vi "SaveWfmTxtNEW (SubVI).vi"(8 "error in":errorcluster, 11 "АЧХ":cluster{dbl[], dbl[]}[](graph) caption="XY Graph - Light") -> (0 "error out":errorcluster)   [LabVIEW 2017]
uses:
  <vilib>/Utility/file.llb/Write Delimited Spreadsheet (DBL).vi
panel:
  out "output array":dbl[][](array[numeric])
  out "Array":dbl[][](array[numeric])
  out "dt":dbl[](array[numeric])
  out "Y":dbl[](array[numeric])
  in  "Osc":waveform(dbl)[](graph)=[{"t0"=timestamp(0 s since 1904-01-01), "dt"=0.0002500000118743628, "Y"=array[20608 elements]}, {"t0"=timestamp(0 s since 1904-01-01), "dt"=0.0002500000118743628, "Y"=array[20608 elements]}, {"t0"=timestamp(0 s since 1904-01-01), "dt"=0.0002500000118743628, "Y"=array[20608 elements]}, {"t0"=timestamp(0 s since 1904-01-01), "dt"=0.0002500000118743628, "Y"=array[20608 elements]}] caption="Осциллограмма"
  # "Сохранение данных"
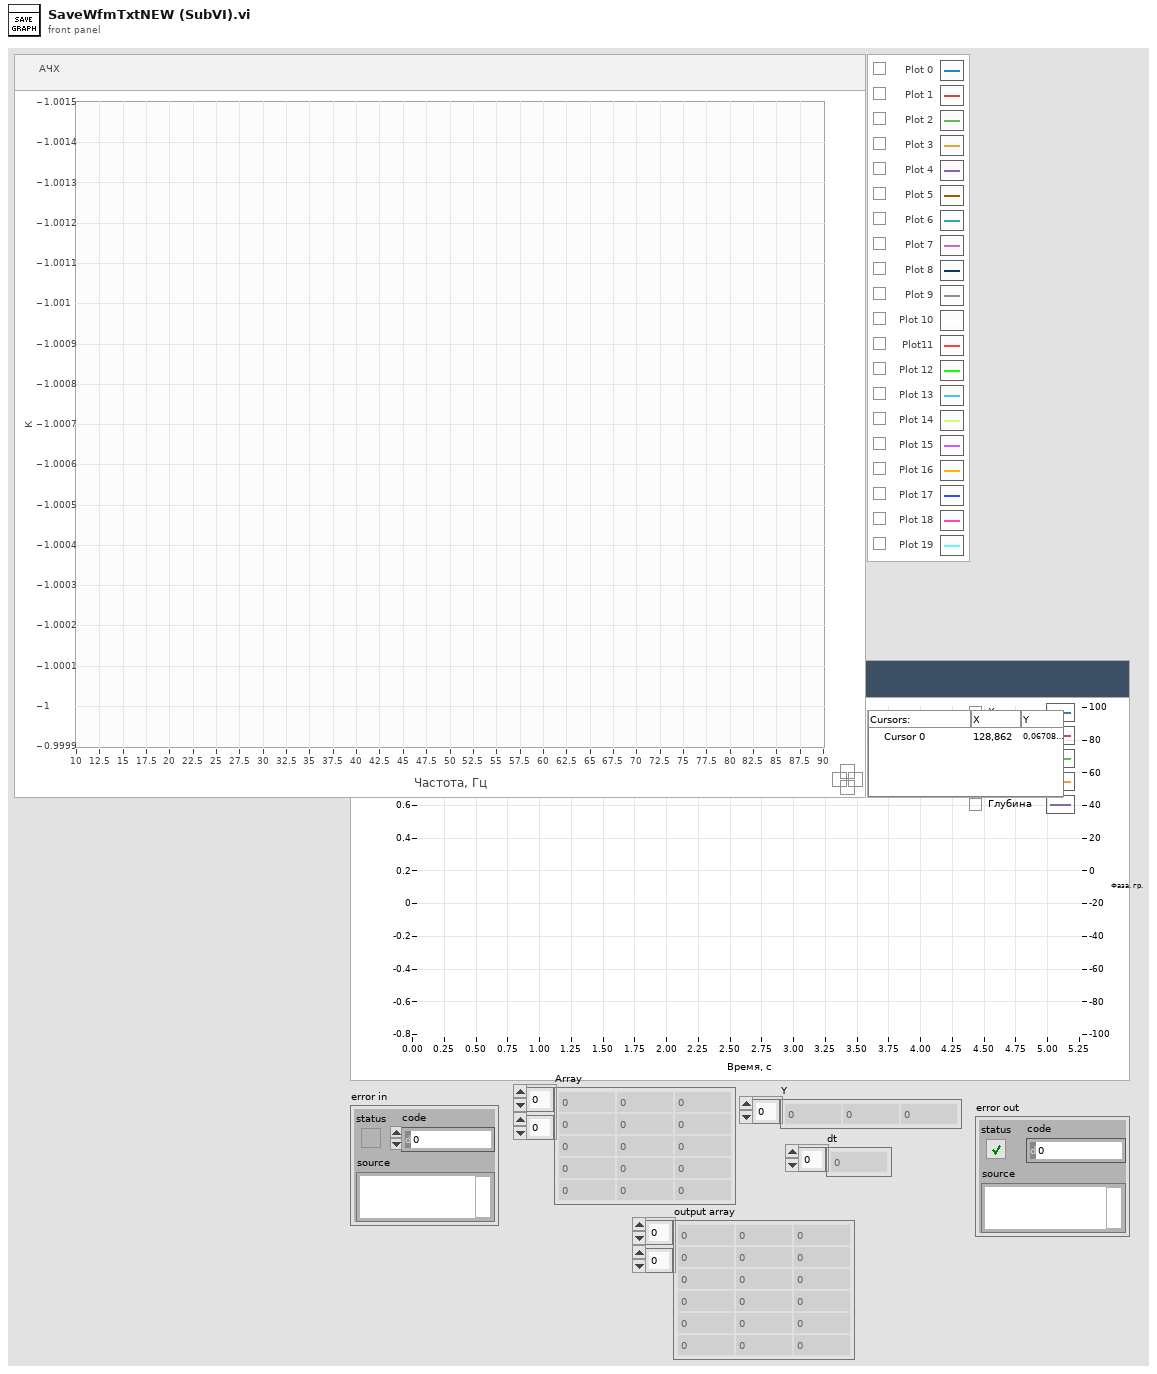
[diagram p1: front panel]
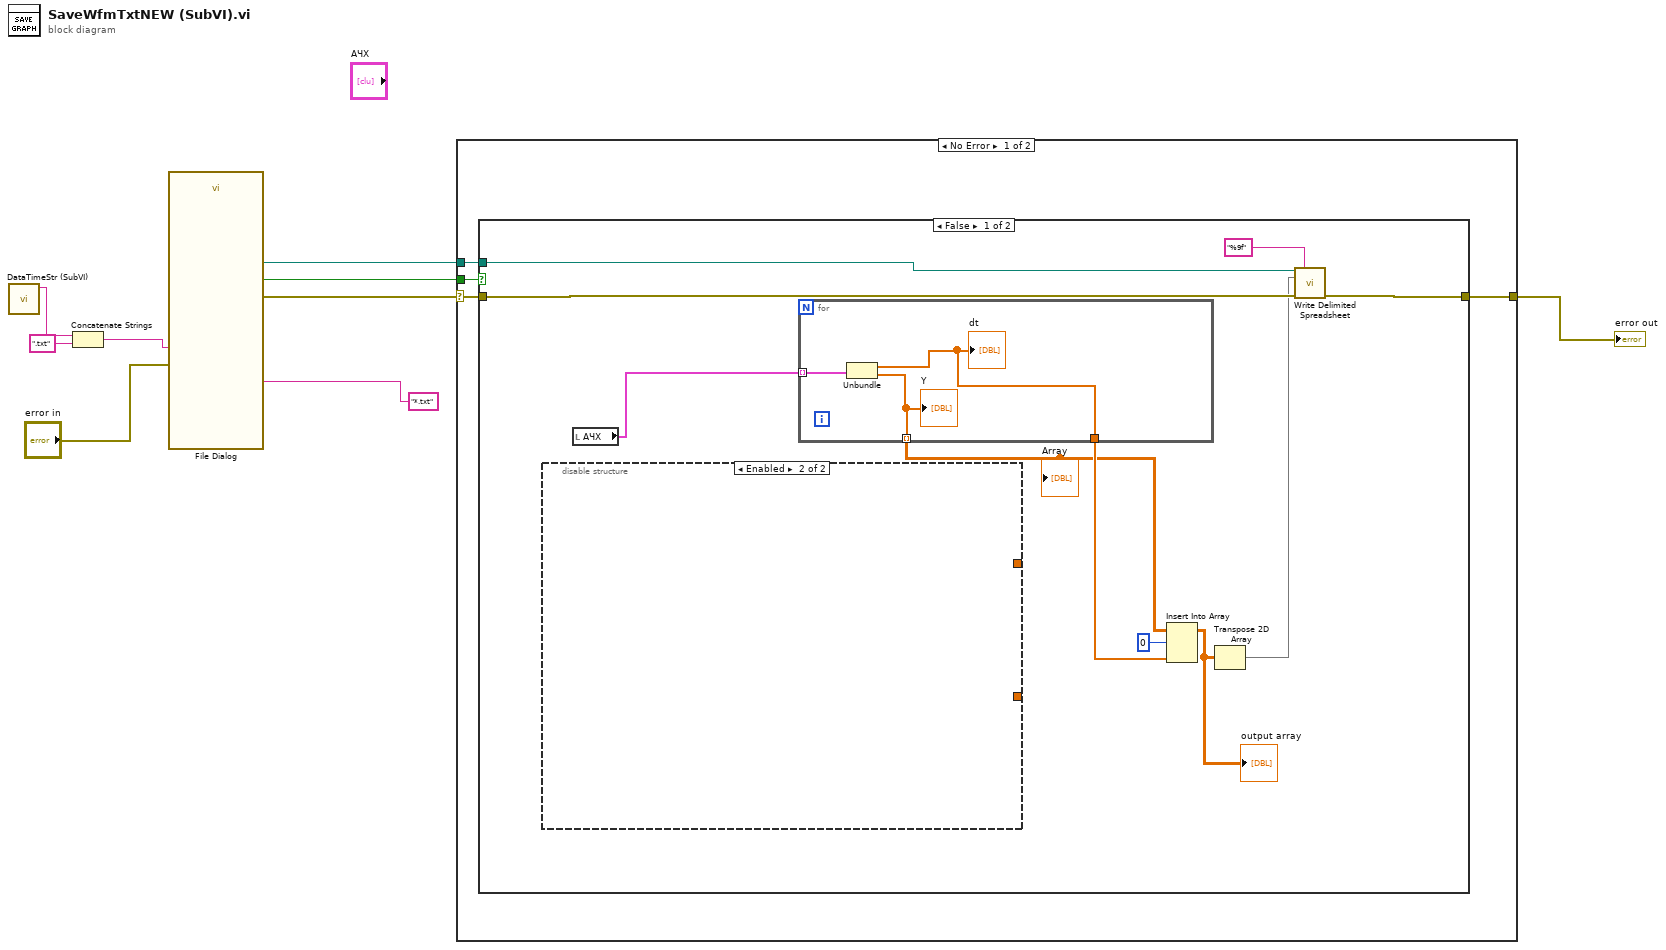
[diagram p0: block diagram]
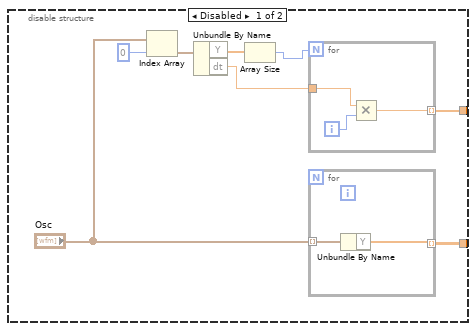
[diagram p2: hidden frame]
diagram:
  n1 = call "DataTimeStr (SubVI).vi"() -> ("DataTimeStr"=w4:string)  [unwired: 11 in]
  n2 = Concatenate Strings(w4, ".txt" ("string")) -> (w2:string)
  n3 = call "File Dialog"("default name"=w2, "error in"="error in", "pattern (all files)"="*.txt") -> ("selected path"=w9:path, "cancelled"=w7:bool, "error out"=w6:errorcluster)  [unwired: 9 in, 1 out]
  n4 = case shown="No Error" w6 {
    selector: w6 -> [w11 w41]
    tunnel: w9 -> [w13 _]
    tunnel: w7 -> [w12 _]
    tunnel: [w10 w41] -> w5
    frame No Error {
      n5 = case shown="False" w12 {
        tunnel: w13 -> [w21 _]
        tunnel: w11 -> [w20 w40]
        tunnel: [w19 w40] -> w10
        frame False {
          n6 = disable-structure shown="Enabled" {
            disable-tunnel: [w25 _] -> _
            disable-tunnel: [w24 _] -> _
            frame Disabled {
              n7 = Index Array(array="Osc", index=0) -> (element=w29:waveform(dbl))
              n8 = Unbundle By Name(w29) -> ("Y"=w28:dbl[], "dt"=w26:dbl)
              n9 = Array Size(array=w28) -> (size(s)=w27:i32)
              n10 = for {
                N: w27 -> [_]
                tunnel: w26 -> [w33]
                tunnel: [w32] -> w24 mode=indexing
                i -> [w34]
                n11 = Multiply(x=w33, y=w34) -> (x*y=w32:dbl)
              }
              n12 = for {
                tunnel: "Osc" -> [w36] mode=indexing
                tunnel: [w35] -> w25 mode=indexing
                n13 = Unbundle By Name(w36) -> ("Y"=w35:dbl[])
              }
            }
            frame Enabled {
            }
          }
          n14 = local read "АЧХ"() -> (w16:cluster{dbl[], dbl[]}[])
          n15 = for {
            tunnel: w16 -> [w37] mode=indexing
            tunnel: [w39] -> w15
            tunnel: [w38] -> w14 mode=indexing
            n16 = Unbundle(w37) -> (w39:dbl[], w38:dbl[])
            "Y" <- w38
            "dt" <- w39
          }
          "Array" <- w14
          n17 = Insert Into Array(array=w14, index (row)=0, new element=w15) -> (w18:dbl[][])  [unwired: 1 in]
          "output array" <- w18
          n18 = Transpose 2D Array(2D array=w18) -> (transposed array=w17:dbl[][])
          n19 = call-poly <vilib>:"Write Delimited Spreadsheet.vi"("file path (dialog if empty)"=w21, "format (%.3f)"="%9f", "2D data"=w17, "error in (no error)"=w20) -> ("error out"=w19:errorcluster)  [unwired: 10 in, 1 out]
        }
        frame True {
        }
      }
    }
    frame Error {
    }
  }
  "error out" <- w5
